vi "SetValueByItemTagArray.vi"(0 "VI Reference In":refnum<vi>, 2 "delimiter (>>)":string=">>", 5 "Control Path":string, 7 "Item Tags Array":string[](array[string]), 11 "Error In":errorcluster) -> (4 "VI Reference Out":refnum<vi>, 15 "Error Out":errorcluster)   [LabVIEW 2016, in "Drona.lvlib" / "ControlValue.lvlib" / "StimulusTree.lvlib"]
doc: "Sets value(signaling) for the multi-select tree control whose item tags are specified as an array. \n\nThe input control name is given as a string , incase of path, use delimiters inbetween the path."
uses:
  StimulusTree.lvlib
  <vilib>/Utility/error.llb/Error Cluster From Error Code.vi
  <vilib>/ErrorRing/Error Ring.xnode
  Drona.lvlib
  Get/GetControlRef/GetControlRef.lvlib
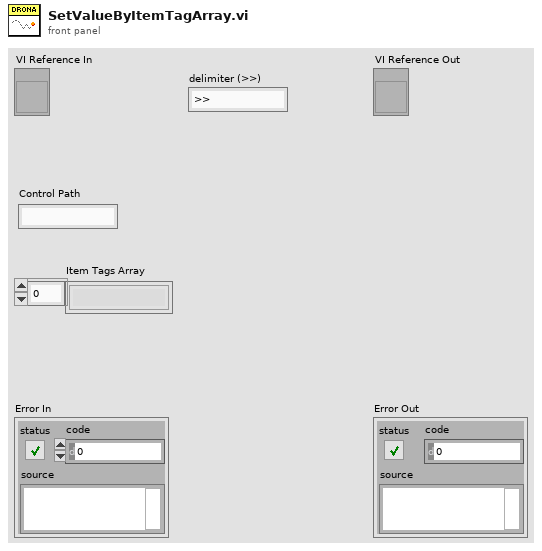
[diagram p1: front panel]
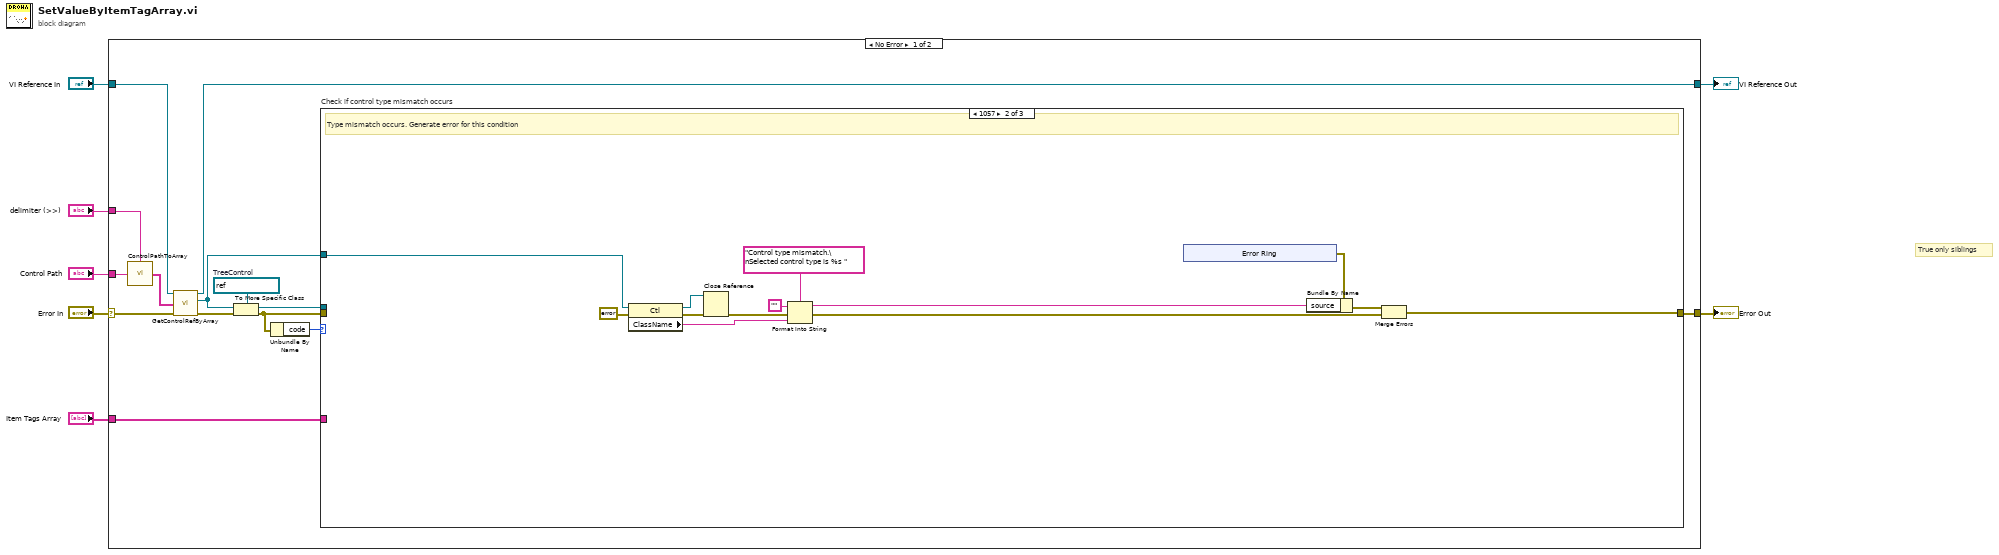
[diagram p0: block diagram]
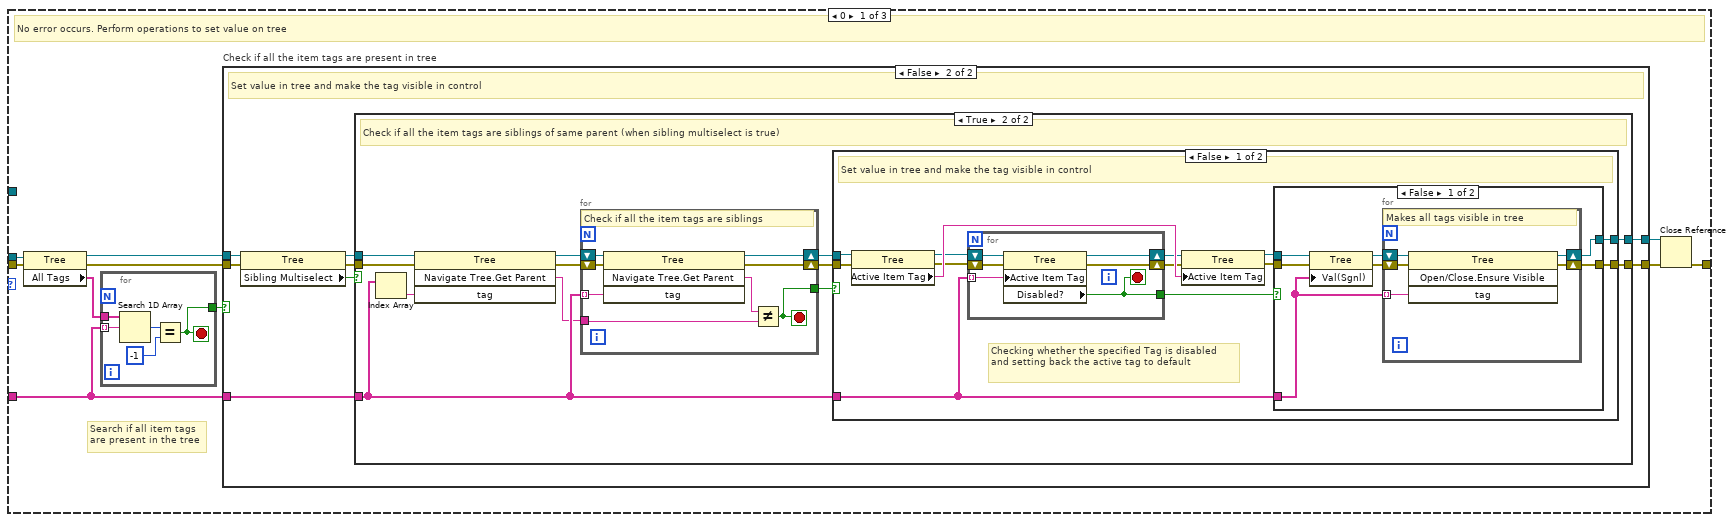
[diagram p2: hidden frame]
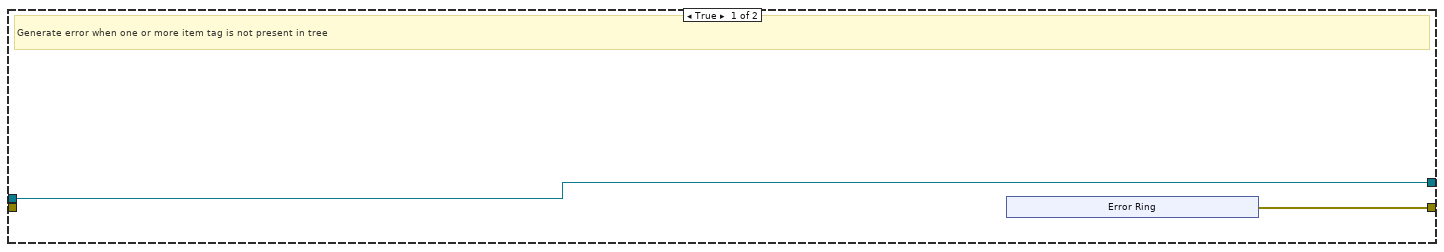
[diagram p3: hidden frame]
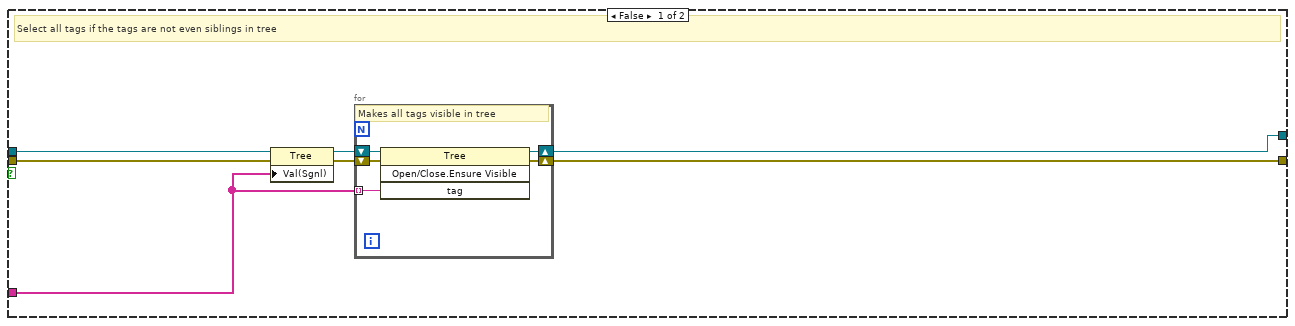
[diagram p4: hidden frame]
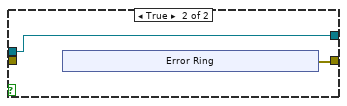
[diagram p5: hidden frame]
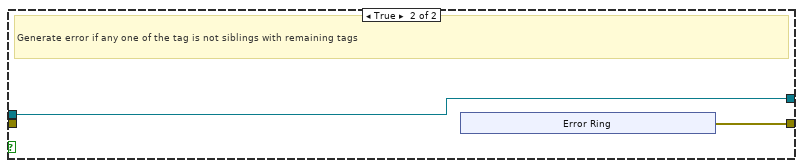
[diagram p6: hidden frame]
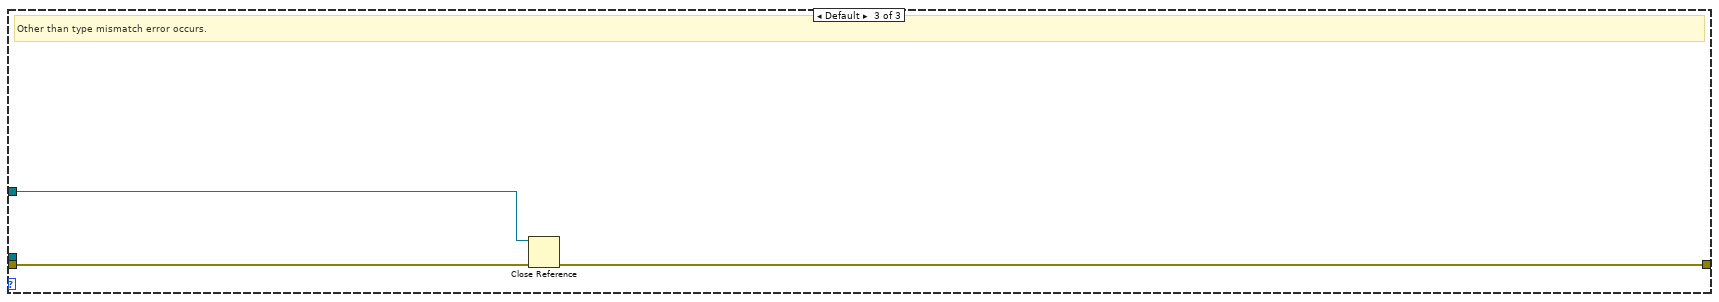
[diagram p7: hidden frame]
diagram:
  # "True only siblings"
  n1 = case shown="No Error" "Error In" {
    selector: "Error In" -> [w18 w151]
    tunnel: [w8 w151] -> w6
    tunnel: "VI Reference In" -> [w17 w150]
    tunnel: "Control Path" -> [w20 _]
    tunnel: [w14 w150] -> w3
    tunnel: "delimiter (>>)" -> [w19 _]
    tunnel: "Item Tags Array" -> [w13 _]
    frame No Error {
      w21 = refnum<vi> refnum  # TreeControl
      n2 = call "ControlPathToArray.vi"("Control Name"=w20, "delimiter (>>)"=w19) -> ("Control Path"=w16:string[])
      n3 = call "GetControlRefByArray.vi"("VI Reference In"=w17, "Control Path"=w16, "error In"=w18) -> ("VI Reference Out"=w14:refnum<vi>, "Ctl Refnum"=w10:refnum<vi>, "error out"=w15:errorcluster)  [unwired: 10 in]
      n4 = To More Specific Class(target class=w21, reference=w10, error in=w15) -> (specific class reference=w11:refnum<vi>, error out=w12:errorcluster)
      n5 = Unbundle By Name(w12) -> ("code"=w9:i32)
      n6 = case "Check if control type mismatch occurs" shown="1057" w9 {
        tunnel: [w31 w131 w148] -> w8
        tunnel: w11 -> [w26 _ _]
        tunnel: w13 -> [w23 _ _]
        tunnel: w10 -> [_ w141 w147]
        tunnel: w12 -> [w30 _ w149]
        frame 0 {
          # "Search if all item tags \nare present in the tree"
          # "No error occurs. Perform operations to set value on tree"
          n7 = property class="Tree"(reference=w26, error in=w30) -> (reference out=w25:refnum<vi>, error out=w27:errorcluster, "All Tags"=w24:string[])
          n8 = for {
            tunnel: w24 -> [w36]
            tunnel: w23 -> [w35] mode=indexing
            tunnel: [w32] -> w22
            stop <- w32 stop-if-true
            n9 = Search 1D Array(1D array=w36, element=w35) -> (index of element=w34:i32)  [unwired: 1 in]
            n10 = Equal?(x=w34, y=-1) -> (x = y?=w32:bool)
          }
          n11 = case "Check if all the item tags are present in tree" shown="False" w22 {
            tunnel: [w37 w50] -> w29
            tunnel: [w38 w49] -> w28
            tunnel: w27 -> [_ w51]
            tunnel: w25 -> [w38 w46]
            tunnel: w23 -> [_ w48]
            frame True {
              # "Generate error when one or more item tag is not present in tree"
              n12 = xnode "Error Ring"() -> ("error out"=w37:errorcluster)
            }
            frame False {
              # "Set value in tree and make the tag visible in control"
              n13 = property class="Tree"(reference=w46, error in=w51) -> (reference out=w44:refnum<vi>, error out=w47:errorcluster, "Sibling Multiselect"=w45:bool)
              n14 = case shown="True" w45 {
                tunnel: [w57 w75] -> w50
                tunnel: [w55 w74] -> w49
                tunnel: w48 -> [w54 w70]
                tunnel: w47 -> [w53 w73]
                tunnel: w44 -> [w52 w71]
                frame False {
                  # "Select all tags if the tags are not even siblings in tree"
                  n15 = property class="Tree"(reference=w52, error in=w53, "Val(Sgnl)"=w54) -> (reference out=w56:refnum<vi>, error out=w58:errorcluster)
                  n16 = for {
                    shift-right: [w62] -> w57
                    shift-left: w58 -> [w63]
                    shift-right: [w60] -> w55
                    shift-left: w56 -> [w61]
                    tunnel: w54 -> [w59] mode=indexing
                    # "Makes all tags visible in tree"
                    n17 = invoke class="Tree" method="Open/Close.Ensure Visible"(reference=w61, error in=w63, "tag"=w59) -> (reference out=w60:refnum<vi>, error out=w62:errorcluster)  [unwired: 1 in, 2 out]
                  }
                }
                frame True {
                  # "Check if all the item tags are siblings of same parent (when sibling multiselect is true)"
                  n18 = Index Array(array=w70) -> (element=w69:string)  [unwired: 1 in]
                  n19 = invoke class="Tree" method="Navigate Tree.Get Parent"(reference=w71, error in=w73, "tag"=w69) -> (reference out=w64:refnum<vi>, error out=w72:errorcluster, "Navigate Tree:Get Parent"=w68:string)  [unwired: 1 in, 1 out]
                  n20 = for {
                    tunnel: w70 -> [w126] mode=indexing
                    shift-right: [w124] -> w66
                    shift-left: w72 -> [w127]
                    shift-right: [w125] -> w65
                    shift-left: w64 -> [w128]
                    tunnel: w68 -> [w122]
                    tunnel: [w121] -> w67
                    stop <- w121 stop-if-true
                    # "Check if all the item tags are siblings"
                    n21 = invoke class="Tree" method="Navigate Tree.Get Parent"(reference=w128, error in=w127, "tag"=w126) -> (reference out=w125:refnum<vi>, error out=w124:errorcluster, "Navigate Tree:Get Parent"=w123:string)  [unwired: 1 in, 1 out]
                    n22 = Not Equal?(x=w123, y=w122) -> (x != y?=w121:bool)
                  }
                  n23 = case shown="False" w67 {
                    tunnel: [w88 w114] -> w75
                    tunnel: [w87 w115] -> w74
                    tunnel: w70 -> [w77 _]
                    tunnel: w66 -> [w81 _]
                    tunnel: w65 -> [w80 w115]
                    frame False {
                      # "Checking whether the specified Tag is disabled and setting back the active tag to default"
                      # "Set value in tree and make the tag visible in control"
                      n24 = property class="Tree"(reference=w80, error in=w81) -> (reference out=w85:refnum<vi>, error out=w84:errorcluster, "Active Item Tag"=w86:string)
                      n25 = for {
                        tunnel: w77 -> [w94] mode=indexing
                        tunnel: [w93] -> w76
                        shift-right: [w92] -> w83
                        shift-left: w84 -> [w91]
                        shift-right: [w90] -> w82
                        shift-left: w85 -> [w89]
                        stop <- w93 stop-if-true
                        n26 = property class="Tree"(reference=w89, error in=w91, "Active Item Tag"=w94) -> (reference out=w90:refnum<vi>, error out=w92:errorcluster, "Disabled?"=w93:bool)
                      }
                      n27 = property class="Tree"(reference=w82, error in=w83, "Active Item Tag"=w86) -> (reference out=w79:refnum<vi>, error out=w78:errorcluster)
                      n28 = case shown="False" w76 {
                        tunnel: [w100 w107] -> w88
                        tunnel: [w98 w108] -> w87
                        tunnel: w77 -> [w97 _]
                        tunnel: w78 -> [w96 _]
                        tunnel: w79 -> [w95 w108]
                        frame False {
                          n29 = property class="Tree"(reference=w95, error in=w96, "Val(Sgnl)"=w97) -> (reference out=w99:refnum<vi>, error out=w101:errorcluster)
                          n30 = for {
                            shift-right: [w105] -> w100
                            shift-left: w101 -> [w106]
                            shift-right: [w103] -> w98
                            shift-left: w99 -> [w104]
                            tunnel: w97 -> [w102] mode=indexing
                            # "Makes all tags visible in tree"
                            n31 = invoke class="Tree" method="Open/Close.Ensure Visible"(reference=w104, error in=w106, "tag"=w102) -> (reference out=w103:refnum<vi>, error out=w105:errorcluster)  [unwired: 1 in, 2 out]
                          }
                        }
                        frame True {
                          n32 = xnode "Error Ring"() -> ("error out"=w107:errorcluster)
                        }
                      }
                    }
                    frame True {
                      # "Generate error if any one of the tag is not siblings with remaining tags"
                      n33 = xnode "Error Ring"() -> ("error out"=w114:errorcluster)
                    }
                  }
                }
              }
            }
          }
          n34 = Close Reference(reference=w28, error in (no error)=w29) -> (error out=w31:errorcluster)
        }
        frame 1057 {
          # "Type mismatch occurs. Generate error for this condition"
          n35 = property class="Ctl"(reference=w141, error in=errorcluster {"status"=FALSE, "code"=0, "source"=""} ("error out")) -> (reference out=w129:refnum<vi>, error out=w140:errorcluster, "ClassName"=w137:string)
          n36 = Close Reference(reference=w129, error in (no error)=w140) -> (error out=w130:errorcluster)
          n37 = Format Into String(format string="Control type mismatch.\nSelected control type is %s ", initial string="", error in=w130, w137) -> (resulting string=w134:string, error out=w132:errorcluster)
          n38 = xnode "Error Ring"() -> ("error out"=w135:errorcluster)
          n39 = Bundle By Name(cluster=w135, "source"=w134) -> (w133:errorcluster)
          n40 = Merge Errors(w133, w132) -> (w131:errorcluster)
        }
        frame Default {
          # "Other than type mismatch error occurs."
          n41 = Close Reference(reference=w147, error in (no error)=w149) -> (error out=w148:errorcluster)
        }
      }
    }
    frame Error {
    }
  }
  "Error Out" <- w6
  "VI Reference Out" <- w3
